vi "niSwitch Close gRPC Session.vi"(8 "error in":errorcluster, 11 "session factory in":refnum<class "Session Factory.lvclass">) -> (0 "error out":errorcluster)   [LabVIEW 2021, in "Session Management niSwitch.lvlib" / "Session Factory.lvclass"]
doc: "Closes the session specified in <b>session factory in</b> and deallocates the resources that NI-Switch reserved."
uses:
  Session Factory.lvclass
  NI Switch Client/RPC Messages/niswitch_grpc_CloseRequest.ctl
  NI Switch Client/RPC Messages/nidevice_grpc_Session.ctl
  NI Switch Client/RPC Messages/nidevice_grpc_Session_session/nidevice_grpc_Session_session.lvclass
  Session Factory.lvclass/Session Factory.ctl
  NI Switch Client/NI Switch Client.lvlib
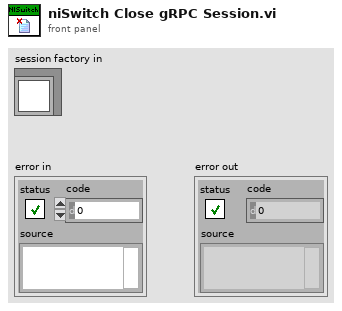
[diagram p1: front panel]
types:
  T1 = typedef "NI Switch Client.lvlib/niswitch_grpc_CloseRequest.ctl" = cluster{"vi":T2}
  T2 = typedef "NI Switch Client.lvlib/nidevice_grpc_Session.ctl" = cluster{"nidevice_grpc_Session_session":refnum<class "nidevice_grpc_Session_session.lvclass">}
  T3 = typedef "grpc-lvsupport-release.lvlib/grpcId.ctl" = u64
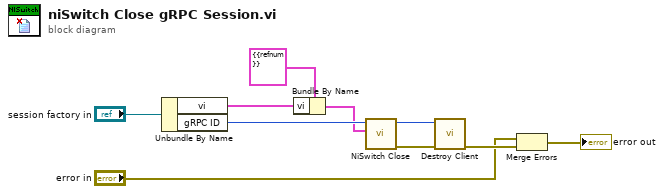
[diagram p0: block diagram]
diagram:
  n1 = Unbundle By Name("session factory in") -> ("vi"=w9:T2, "gRPC ID"=w10:T3)
  n2 = Bundle By Name(cluster=T1 {"vi"={"nidevice_grpc_Session_session"=refnum}} ("Request Data"), "vi"=w9) -> (w7:T1)
  n3 = call "NiSwitch Close.vi"("Request Data"=w7, "gRPC ID"=w10) -> ("error out"=w5:errorcluster, "gRPC ID out"=w6:T3)  [unwired: 7 in, 1 out]
  n4 = call "Destroy Client.vi"("error in"=w5, "gRPC ID"=w6) -> ("error out"=w4:errorcluster)  [unwired: 9 in]
  n5 = Merge Errors("error in", w4) -> (→"error out":errorcluster)
